vi "Convert Argument Representation.vi"(10 "error argument string":string) -> (1 "Data":string[](array[string]), 2 "Arguments":string[](array[string]), 3 "Formatted Argument":string)   [LabVIEW 2019, in "Error Generation.lvlib"]
doc: "Convert a argument sting from the format\n\nargument name = argument data\nargument name = argument data\n\nto the format\n\n< b >argument name< /b >\nargument data\n< b >argument name< /b >\nargument data\n\nEmpty data are allowed.\nWhen there is no \"=\" input string equal to output string.\n- - -\nCopyright (c) 2023, Merecs Engineering GmbH"
uses:
  Error Generation.lvlib
panel:
  out "error out":errorcluster
  # "Connector Pane"
  # "Locals"
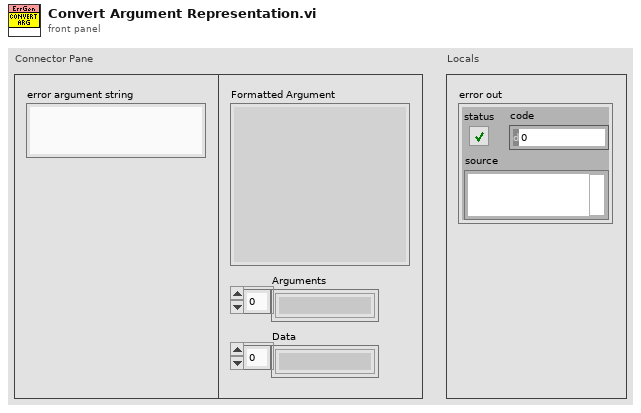
[diagram p1: front panel]
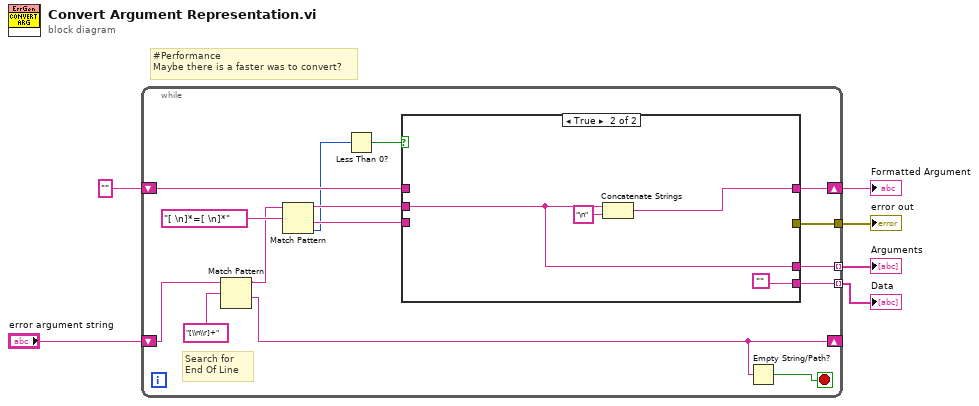
[diagram p0: block diagram]
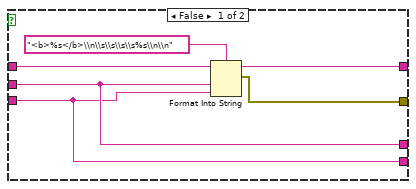
[diagram p2: hidden frame]
diagram:
  # "#Performance\nMaybe there is a faster was to convert?"
  n1 = while {
    shift-right: [w12] -> _
    shift-left: "error argument string" -> [w19]
    shift-right: [w15] -> w4
    shift-left: "" ("error argument string (arg>>data\\n)") -> [w14]
    tunnel: [w9] -> w3 mode=indexing
    tunnel: [w8] -> w2 mode=indexing
    tunnel: [w7] -> w1
    stop <- w13 stop-if-true
    # "Search for End Of Line"
    n2 = Match Pattern(string=w19, regular expression="[\\n\\r]+") -> (before substring=w18:string, after substring=w12:string)  [unwired: 1 in, 2 out]
    n3 = Match Pattern(string=w18, regular expression="[ \n]*=[ \n]*") -> (before substring=w17:string, after substring=w16:string, offset past match=w11:i32)  [unwired: 1 in, 1 out]
    n4 = Less Than 0?(x=w11) -> (x < 0?=w10:bool)
    n5 = case shown="True" w10 {
      tunnel: [w27 w31] -> w15
      tunnel: w17 -> [w24 w29]
      tunnel: w16 -> [w23 _]
      tunnel: w14 -> [w25 _]
      tunnel: [w24 w29] -> w9
      tunnel: [w23 "" ("error argument string")] -> w8
      tunnel: [w22 _] -> w7
      frame False {
        n6 = Format Into String(format string="<b>%s</b>\\n\\s\\s\\s\\s%s\\n\\n", initial string=w25, w24, w23) -> (resulting string=w27:string, error out=w22:errorcluster)  [unwired: 1 in]
      }
      frame True {
        n7 = Concatenate Strings(w29, "\n" ("string")) -> (w31:string)
      }
    }
    n8 = Empty String/Path?(string/path=w12) -> (empty?=w13:bool)
  }
  "Formatted Argument" <- w4
  "Arguments" <- w3
  "Data" <- w2
  "error out" <- w1
